vi "Copy .LLB to NI VeriStand dir.vi"(5 "Files Generated by Build":path[](array[path]), 6 "Top Level/Always Included VIs":path[](array[path]), 7 "Destination Path":path, 8 "error in (no error)":errorcluster, 9 "Target Name":string, 10 "Build Specification Name":string, 11 "Project Path":path) -> (0 "error out":errorcluster)   [LabVIEW 2024]
doc: "This VI is called after each run of a build specification. The VI will copy the generated LLB (Engine or System Explorer) into the VeriStand Custom Device folder (...\\Documents\\National Instruments\\NI VeriStand 2013...)."
uses:
  <vilib>/Utility/sysdir.llb/System Directory Type.ctl
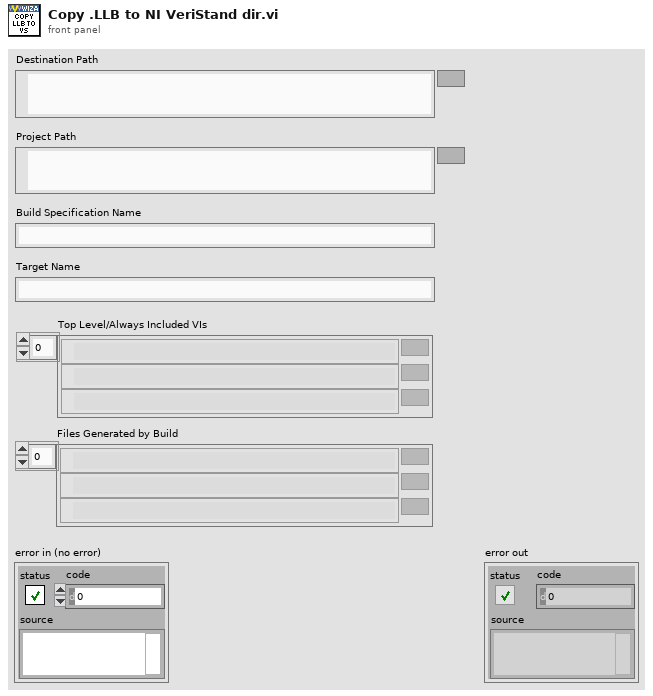
[diagram p1: front panel]
types:
  T1 = typedef "System Directory Type.ctl" = i32
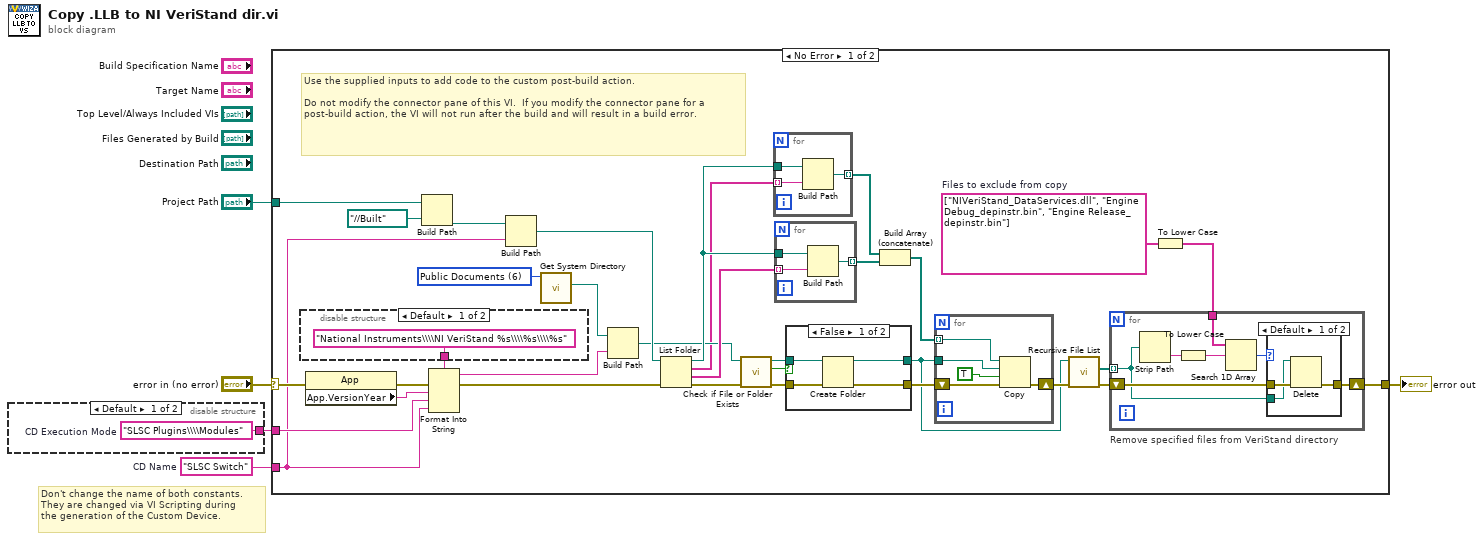
[diagram p0: block diagram]
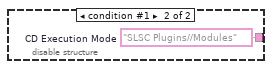
[diagram p2: hidden frame]
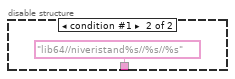
[diagram p3: hidden frame]
diagram:
  w2 = "SLSC Switch"  # CD Name
  # "Don't change the name of both constants.\nThey are changed via VI Scripting during\nthe generation of the Custom Device."
  n1 = disable-structure shown="Default" {
    disable-tunnel: [w6 w7] -> w3
    frame condition #0 (active) {
      w6 = "SLSC Plugins\\\\Modules"  # CD Execution Mode
    }
    frame condition #1 {
      w7 = "SLSC Plugins//Modules"  # CD Execution Mode
    }
  }
  n2 = case shown="No Error" "error in (no error)" {
    selector: "error in (no error)" -> [w22 w71]
    tunnel: [w9 w71] -> w1
    tunnel: "Project Path" -> [w18 _]
    tunnel: w3 -> [w23 _]
    tunnel: w2 -> [w20 _]
    frame No Error {
      w15 = string[] ["NIVeriStand_DataServices.dll", "Engine Debug_depinstr.bin", "Engine Release_depinstr.bin"]  # Files to exclude from copy
      w28 = T1 6 items=["User Home"=0, "User Desktop"=1, "User Documents"=2, "User Application Data"=3, "User Preferences"=4, "User Temporary"=5, "Public Documents"=6, "Public Application Data"=7, "Public Preferences"=8, "Public Cache"=13, "System Core Libraries"=9, "System Installed Libraries"=10, "Application Files"=11, "Boot Volume Root"=12] ("system directory type")
      # "Use the supplied inputs to add code to the custom post-build action.\n\nDo not modify the connector pane of this VI.  If you modify the connector pane for a post-build action, the VI will not run after the build and will result in a build error."
      n3 = disable-structure shown="Default" {
        disable-tunnel: ["National Instruments\\\\NI VeriStand %s\\\\%s\\\\%s" ("name or relative path") "lib64//niveristand%s//%s//%s" ("name or relative path")] -> w25
        frame condition #0 (active) {
        }
        frame condition #1 {
        }
      }
      n4 = property class="App"(error in=w22) -> (error out=w27:errorcluster, "App.VersionYear"=w26:string)  [unwired: 1 in, 1 out]
      n5 = Build Path(base path=w18, name or relative path=path "../../Built") -> (appended path=w8:path)
      n6 = Format Into String(format string=w25, error in=w27, w26, w23, w20) -> (resulting string=w30:string, error out=w21:errorcluster)  [unwired: 1 in]
      n7 = Build Path(base path=w8, name or relative path=w20) -> (appended path=w32:path)
      n8 = call <vilib>:"Get System Directory.vi"("system directory type"=w28) -> ("system directory"=w29:path)  [unwired: 10 in]
      n9 = Build Path(base path=w29, name or relative path=w30) -> (appended path=w24:path)
      n10 = List Folder(path=w32, error in=w21) -> (path out=w34:path, filenames=w16:string[], folder names=w35:string[], error out=w31:errorcluster)  [unwired: 2 in]
      n11 = call <vilib>:"Check if File or Folder Exists.vi"("error in (no error)"=w31, "path"=w24) -> ("error out"=w36:errorcluster, "file or folder exists?"=w38:bool, "dup path"=w37:path)  [unwired: 7 in]
      n12 = for {
        tunnel: w16 -> [w69] mode=indexing
        tunnel: w34 -> [w70]
        tunnel: [w68] -> w40 mode=indexing
        n13 = Build Path(base path=w70, name or relative path=w69) -> (appended path=w68:path)
      }
      n14 = for {
        tunnel: w35 -> [w66] mode=indexing
        tunnel: w34 -> [w67]
        tunnel: [w65] -> w33 mode=indexing
        n15 = Build Path(base path=w67, name or relative path=w66) -> (appended path=w65:path)
      }
      n16 = case shown="False" w38 {
        tunnel: w37 -> [w57 w59]
        tunnel: w36 -> [w56 w58]
        tunnel: [w55 w59] -> w10
        tunnel: [w54 w58] -> w17
        frame False {
          n17 = Create Folder(path (use dialog)=w57, error in=w56) -> (created path=w55:path, error out=w54:errorcluster)  [unwired: 1 in, 1 out]
        }
        frame True {
        }
      }
      n18 = Build Array (concatenate)(w40, w33) -> (w39:path[])
      n19 = for {
        tunnel: w39 -> [w61] mode=indexing
        shift-right: [w62] -> w11
        shift-left: w17 -> [w63]
        tunnel: w10 -> [w60]
        n20 = Copy(8:w63, 9:TRUE ("overwrite (F)"), 10:w60, 11:w61) -> (0:w62:errorcluster)  [unwired: 1 in, 2 out]
      }
      n21 = call <vilib>:"Recursive File List.vi"("error in (no error)"=w11, "Folder Path"=w10) -> ("error out"=w14:errorcluster, "All Files in Dir"=w13:path[])  [unwired: 5 in, 3 out]
      n22 = To Lower Case(string=w15) -> (all lower case string=w12:string[])
      n23 = for "Remove specified files from VeriStand directory" {
        shift-right: [w44] -> w9
        shift-left: w14 -> [w46]
        tunnel: w13 -> [w43] mode=indexing
        tunnel: w12 -> [w47]
        n24 = Strip Path(path=w43) -> (name=w49:string)  [unwired: 1 out]
        n25 = To Lower Case(string=w49) -> (all lower case string=w48:string)
        n26 = Search 1D Array(1D array=w47, element=w48) -> (index of element=w45:i32)  [unwired: 1 in]
        n27 = case shown="Default" w45 {
          tunnel: w46 -> [w52 w53]
          tunnel: [w51 w53] -> w44
          tunnel: w43 -> [w50 _]
          frame Default {
            n28 = Delete(path (use dialog)=w50, error in=w52) -> (error out=w51:errorcluster)  [unwired: 3 in, 2 out]
          }
          frame -1 {
          }
        }
      }
    }
    frame Error {
    }
  }
  "error out" <- w1
